vi "Resolve Type From Assembly File.vi"(8 "error in (no error)":errorcluster, 10 "Type Name":string, 11 "AssemblyFile":path) -> (0 "error out":errorcluster, 3 "GetType out":refnum<k24>)   [LabVIEW 2026, in "ToastNotification.lvlib" / "Reflection DotNet.lvlib"]
doc: "Loads a .NET assembly from AssemblyFile and resolves Type Name in that assembly. Supply the fully qualified type name without an assembly suffix. Skips loading and type resolution on incoming error. Releases the temporary assembly reference after the lookup. The caller owns the returned type reference and must release it after use."
uses:
  Reflection DotNet.lvlib
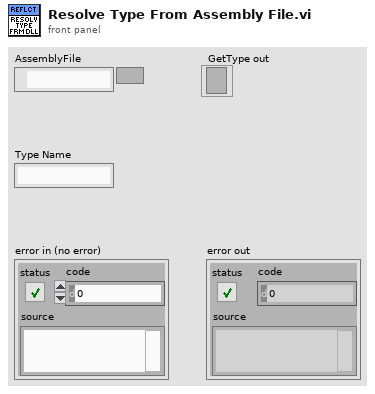
[diagram p1: front panel]
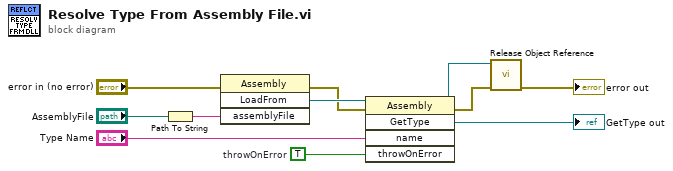
[diagram p0: block diagram]
diagram:
  w4 = TRUE  # throwOnError
  n1 = Path To String(path="AssemblyFile") -> (string=w1:string)
  n2 = invoke class="Assembly" method="LoadFrom"(error in="error in (no error)", "assemblyFile"=w1) -> (error out=w3:errorcluster, "LoadFrom"=w5:refnum<k24>)  [unwired: 2 in, 2 out]
  n3 = invoke class="Assembly" method="GetType"(reference=w5, error in=w3, "name"="Type Name", "throwOnError"=w4) -> (reference out=w8:refnum<k24>, error out=w6:errorcluster, "GetType"=→"GetType out":refnum<k24>)  [unwired: 1 in, 2 out]
  n4 = call "Release Object Reference.vi"("error in"=w6, "object"=w8) -> ("error out"=→"error out":errorcluster)  [unwired: 9 in]
